vi "check Resource Array-Eload.vi"(0 "Resource names":string[](array[string]), 5 "Device current rating":dbl, 7 "Expected current level":dbl, 9 "Mode of operation":T1(ring)=enum."Perform measurement", 11 "error in":errorcluster) -> (4 "Single or ganged configuration":bool, 6 "Single/Master resouce name":string, 8 "Slave resource names":string[](array[string]), 10 "Number of devices used":i32, 15 "error out":errorcluster)   [LabVIEW 2021]
doc: "This vi will scan the resource name array and gives out if configuration is single or ganged, along with that it also checks how many eload are required for running the measurement from device current rating."
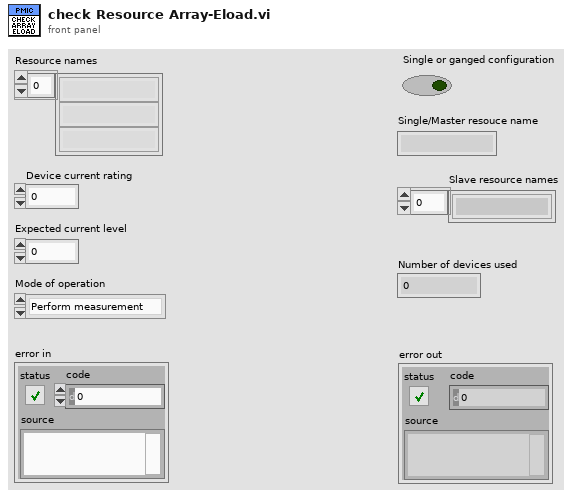
[diagram p1: front panel]
types:
  T1 = enum32{"Power on the DUT", "Perform measurement", "Power off the DUT"}
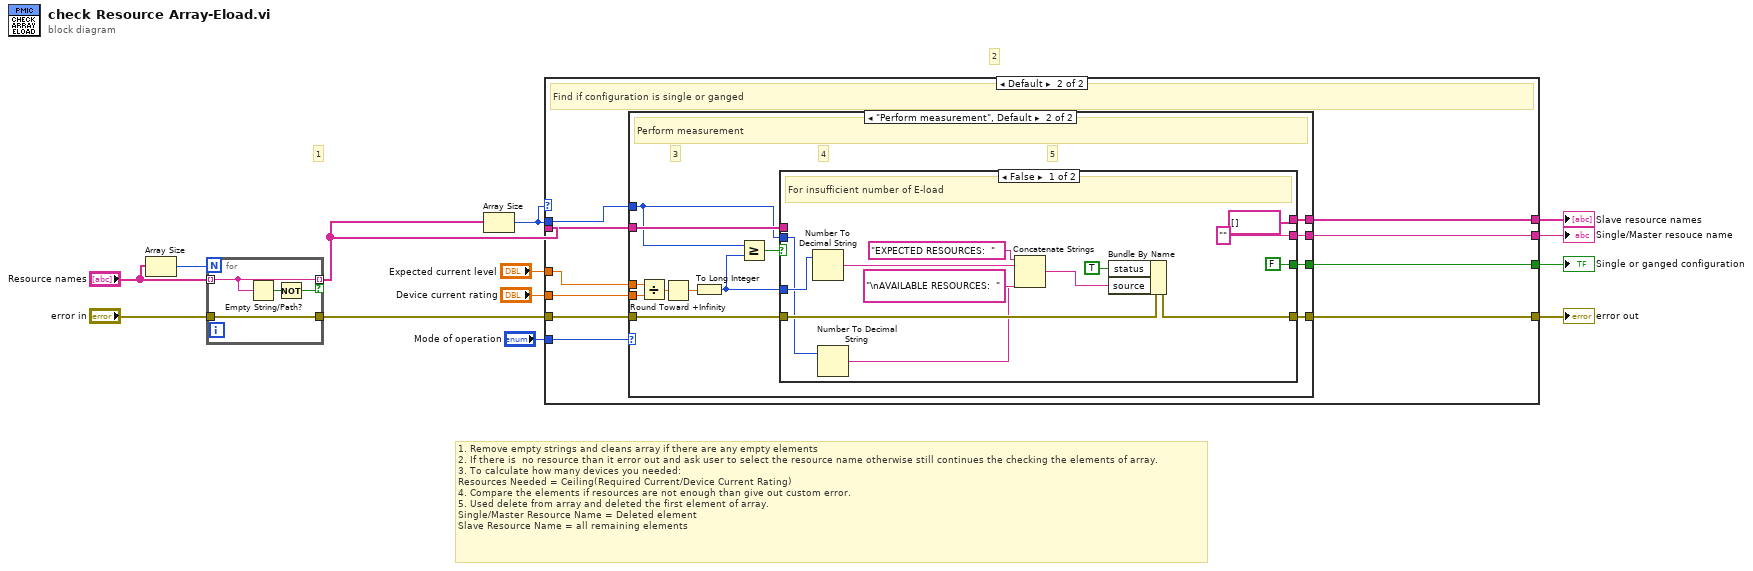
[diagram p0: block diagram]
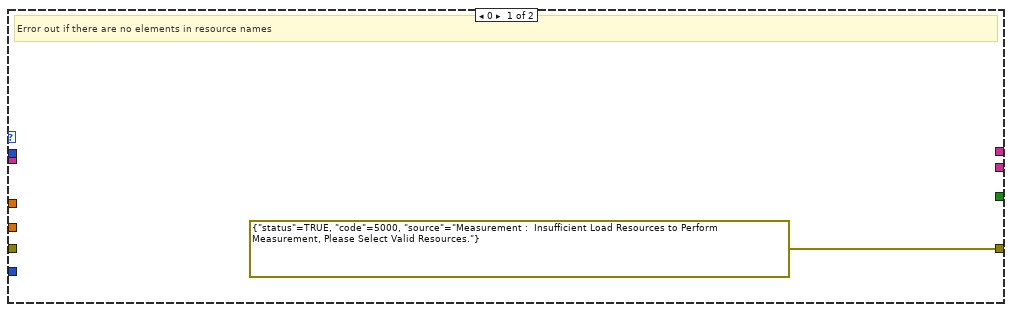
[diagram p2: hidden frame]
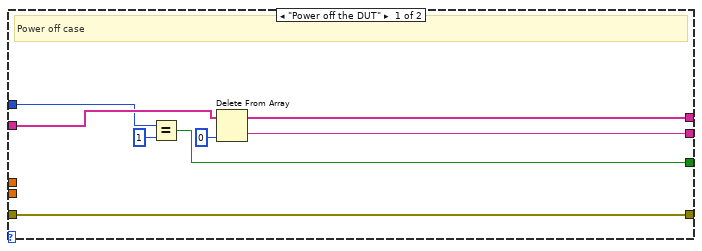
[diagram p3: hidden frame]
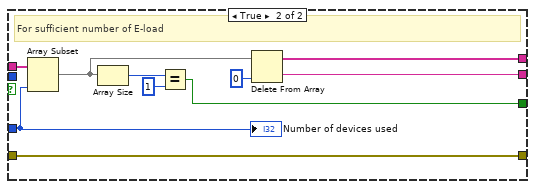
[diagram p4: hidden frame]
diagram:
  # "2"
  # "1"
  # "1. Remove empty strings and cleans array if there are any empty elements\n2. If there is  no resource than it error out and ask user to select the resource name otherwise still continues the checking the elements of array.\n3. To calculate how many devices you needed:\nResources Needed = Ceiling(Required Current/Device Current Rating)\n4. Compare the elements if resources are not enough than give out custom error.\n5. Used delete from array and deleted the first element of array.\nSingle/Master Resource Name = Deleted element\nSlave Resource Name = all remaining elements"
  n1 = Array Size(array="Resource names") -> (size(s)=w10:i32)
  n2 = for {
    N: w10 -> [_]
    tunnel: "Resource names" -> [w16] mode=indexing
    tunnel: "error in" -> [w17]
    tunnel: [w17] -> w9
    tunnel: [w16] -> w8 mode=indexing if=w14
    n3 = Empty String/Path?(string/path=w16) -> (empty?=w15:bool)
    n4 = Not(x=w15) -> (.not. x?=w14:bool)
  }
  n5 = Array Size(array=w8) -> (size(s)=w3:i32)
  n6 = case shown="Default" w3 {
    tunnel: "Device current rating" -> [_ w28]
    tunnel: w9 -> [_ w27]
    tunnel: w8 -> [_ w26]
    tunnel: "Expected current level" -> [_ w25]
    tunnel: [_ w24] -> w6
    tunnel: [_ w23] -> w5
    tunnel: [_ w22] -> w4
    tunnel: w3 -> [_ w21]
    tunnel: [errorcluster {"status"=TRUE, "code"=5000, "source"="Measurement :  Insufficient Load Resources to Perform Measurement, Please Select Valid Resources."} ("error constant") w20] -> w2
    tunnel: "Mode of operation" -> [_ w19]
    frame 0 {
      # "Error out if there are no elements in resource names"
    }
    frame Default {
      # "Find if configuration is single or ganged"
      n7 = case shown="\"Perform measurement\", Default" w19 {
        tunnel: w28 -> [_ w47]
        tunnel: w25 -> [_ w46]
        tunnel: w27 -> [w35 w43]
        tunnel: [w35 w42] -> w20
        tunnel: w26 -> [w32 w41]
        tunnel: [w31 w40] -> w24
        tunnel: [w30 w39] -> w23
        tunnel: [w33 w38] -> w22
        tunnel: w21 -> [w29 w37]
        frame "Power off the DUT" {
          # "Power off case"
          n8 = Equal?(x=w29, y=1) -> (x = y?=w33:bool)
          n9 = Delete From Array(array=w32, index=0) -> (deleted portion=w30:string, array with subset deleted=w31:string[])  [unwired: 1 in]
        }
        frame "Perform measurement", Default {
          # "5"
          # "4"
          # "3"
          # "Perform measurement"
          n10 = Divide(x=w46, y=w47) -> (x/y=w49:dbl)
          n11 = Round Toward +Infinity(x=w49) -> (ceil(x): smallest int >= x=w48:dbl)
          n12 = To Long Integer(number=w48) -> (32bit integer=w45:i32)
          n13 = Greater Or Equal?(x=w37, y=w45) -> (x >= y?=w44:bool)
          n14 = case shown="False" w44 {
            tunnel: w41 -> [_ w68]
            tunnel: w45 -> [w54 w67]
            tunnel: w43 -> [w61 w66]
            tunnel: [w62 w66] -> w42
            tunnel: w37 -> [w53 _]
            tunnel: [string[] [] w65] -> w40
            tunnel: ["" ("String") w64] -> w39
            tunnel: [FALSE w63] -> w38
            frame False {
              # "For insufficient number of E-load"
              n15 = Number To Decimal String(number=w54) -> (decimal integer string=w57:string)  [unwired: 1 in]
              n16 = Number To Decimal String(number=w53) -> (decimal integer string=w56:string)  [unwired: 1 in]
              n17 = Concatenate Strings("EXPECTED RESOURCES:  " ("string"), w57, "\nAVAILABLE RESOURCES:  " ("string"), w56) -> (w60:string)
              n18 = Bundle By Name(cluster=w61, "status"=TRUE, "source"=w60) -> (w62:errorcluster)
            }
            frame True {
              # "For sufficient number of E-load"
              n19 = Array Subset(array=w68, length=w67) -> (w70:string[])  [unwired: 1 in]
              n20 = Array Size(array=w70) -> (size(s)=w72:i32)
              n21 = Equal?(x=w72, y=1) -> (x = y?=w63:bool)
              n22 = Delete From Array(array=w70, index=0) -> (deleted portion=w64:string, array with subset deleted=w65:string[])  [unwired: 1 in]
              "Number of devices used" <- w67
            }
          }
        }
      }
    }
  }
  "Single/Master resouce name" <- w5
  "Slave resource names" <- w6
  "Single or ganged configuration" <- w4
  "error out" <- w2
